vi "Sous_VI_Lanceur.vi"(8 "error in (no error)":errorcluster, 11 "Nb balles":i32) -> (0 "error out":errorcluster)   [LabVIEW 2017]
uses:
  enum_moteur_lanceur.ctl
  enum_distributeur_lanceur.ctl
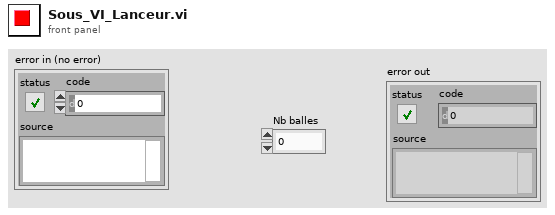
[diagram p1: front panel]
types:
  T1 = typedef "enum_distributeur_lanceur.ctl" = enum16{"Arret", "Marche"}
  T2 = typedef "enum_moteur_lanceur.ctl" = enum16{"distance", "sans_distance", "desactive"}
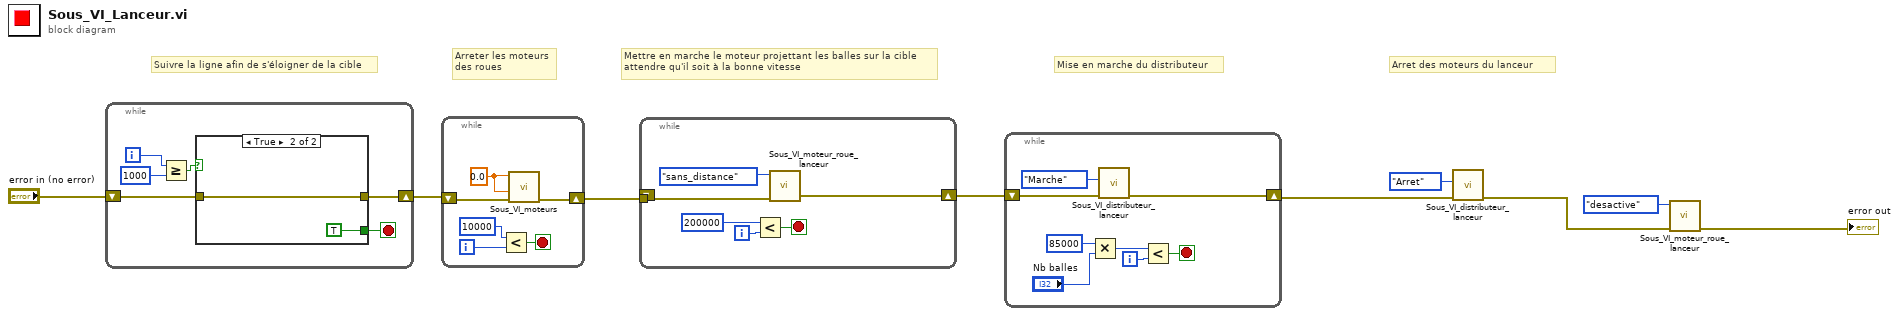
[diagram p0: block diagram]
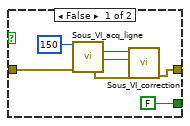
[diagram p2: hidden frame]
diagram:
  # "Arret des moteurs du lanceur"
  # "Mise en marche du distributeur"
  # "Mettre en marche le moteur projettant les balles sur la cible\nattendre qu'il soit à la bonne vitesse"
  # "Arreter les moteurs\ndes roues"
  # "Suivre la ligne afin de s'éloigner de la cible"
  n1 = while {
    shift-right: [w10] -> w7
    shift-left: "error in (no error)" -> [w11]
    i -> [w12]
    stop <- w14 stop-if-true
    n2 = Greater Or Equal?(x=w12, y=1000) -> (x >= y?=w15:bool)
    n3 = case shown="True" w15 {
      tunnel: [FALSE TRUE] -> w14
      tunnel: w11 -> [w19 w23]
      tunnel: [w16 w23] -> w10
      frame False {
        n4 = call "Sous_VI_acq_ligne.vi"("Seuil"=150, "error in (no error)"=w19) -> ("Décalage"=w21:u32, "G/D ?"=w18:bool, "error out"=w17:errorcluster)  [unwired: 8 in, 3 out]
        n5 = call "Sous_VI_correction.vi"("error in (no error)"=w17, "G/D ?"=w18, "Décalage"=w21) -> ("error out"=w16:errorcluster)  [unwired: 8 in]
      }
      frame True {
      }
    }
  }
  n6 = while {
    shift-right: [w25] -> w6
    shift-left: w7 -> [w26]
    i -> [w30]
    stop <- w28 stop-if-true
    w27 = 0.0 ("Moteur Gauche")
    n7 = Less?(x=10000, y=w30) -> (x < y?=w28:bool)
    n8 = call "Sous_VI_moteurs.vi"("error in (no error)"=w26, "Moteur Droit"=w27, "Moteur Gauche"=w27) -> ("error out"=w25:errorcluster)  [unwired: 8 in]
  }
  n9 = while {
    tunnel: w6 -> [w32]
    shift-right: [w31] -> w5
    shift-left: _ -> [_]
    i -> [w36]
    stop <- w34 stop-if-true
    n10 = Less?(x=200000, y=w36) -> (x < y?=w34:bool)
    n11 = call "Sous_VI_moteur_roue_lanceur.vi"("error in (no error)"=w32, "Mode"=enum_moteur_lanceur."sans_distance") -> ("error out"=w31:errorcluster)  [unwired: 9 in]
  }
  n12 = while {
    shift-right: [w37] -> w3
    shift-left: w5 -> [w38]
    i -> [w44]
    stop <- w43 stop-if-true
    n13 = Multiply(x=85000, y="Nb balles") -> (x*y=w40:i32)
    n14 = call "Sous_VI_distributeur_lanceur.vi"("error in (no error)"=w38, "Enum"=enum_distributeur_lanceur."Marche") -> ("error out"=w37:errorcluster)  [unwired: 9 in]
    n15 = Less?(x=w40, y=w44) -> (x < y?=w43:bool)
  }
  n16 = call "Sous_VI_distributeur_lanceur.vi"("error in (no error)"=w3, "Enum"=enum_distributeur_lanceur."Arret") -> ("error out"=w2:errorcluster)  [unwired: 9 in]
  n17 = call "Sous_VI_moteur_roue_lanceur.vi"("error in (no error)"=w2, "Mode"=enum_moteur_lanceur."desactive") -> ("error out"=→"error out":errorcluster)  [unwired: 9 in]
